vi "BIN_PAQ_Concat_PAQ_samples.vi"(7 "Memory TAGs":string[](array[string]), 8 "error in (no error)":errorcluster, 9 "Added samples TAGs":string[](array[string]), 10 "PAQ Samples to ADD":T1, 11 "PAQ Samples IN":T1) -> (0 "error out":errorcluster, 3 "PAQ Samples OUT":T1)   [LabVIEW 2020, in "Sgraph_lib_V1.lvlib" / "DBAL-BIN.lvclass"]
doc: "Andre Koelewijn, 7 mar 2021\n\nThis vi will concatenate PAQ samples based on a PAQ taglist of the samples as it is required for loading in FAMM memory. This routine will add the content based on newest data first. It will subsequenctly expect data chuncks going back in time for every iteration."
uses:
  DBAL-BIN.lvclass
  controls/BIN/BINdata.ctl
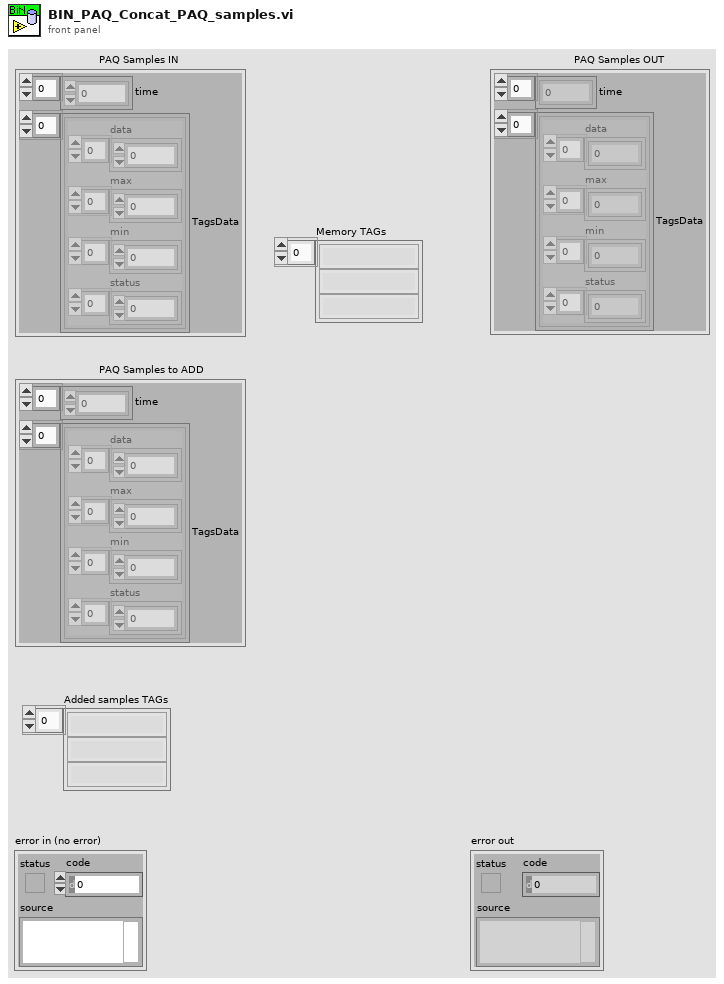
[diagram p1: front panel]
types:
  T1 = typedef "Sgraph_lib_V1.lvlib/DBAL-BIN.lvclass/BINdata.ctl" = cluster{"time":dbl[], "TagsData":cluster{"data":dbl[], "max":dbl[], "min":dbl[], "status":u32[]}[]}
  T2 = cluster{"data":dbl[], "max":dbl[], "min":dbl[], "status":u32[]}[]
  T3 = cluster{"data":dbl[], "max":dbl[], "min":dbl[], "status":u32[]}
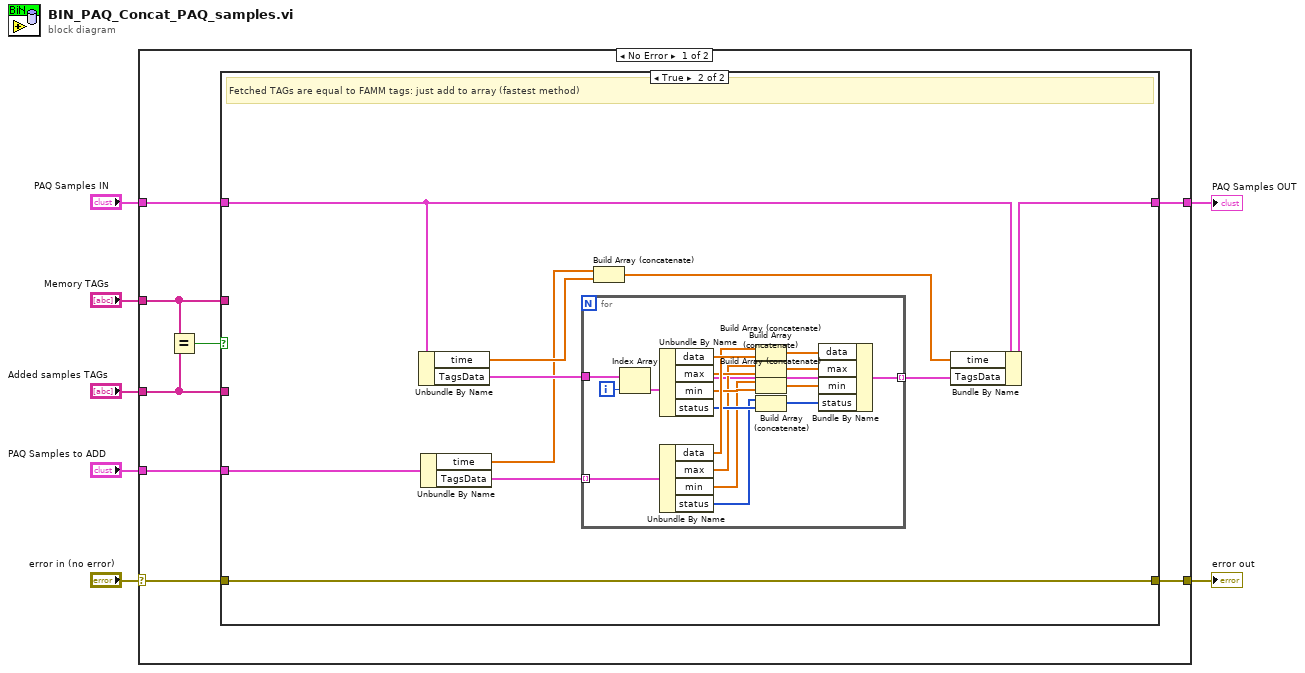
[diagram p0: block diagram]
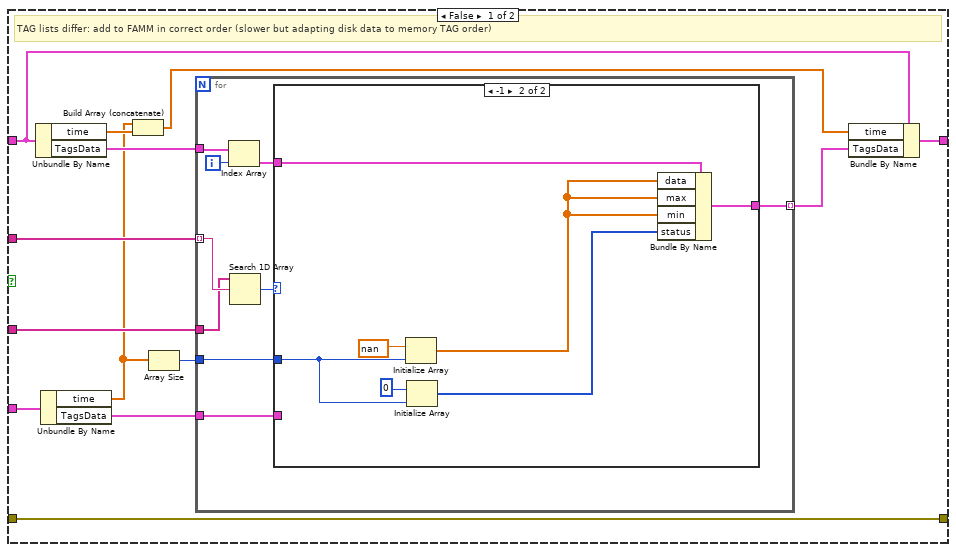
[diagram p2: hidden frame]
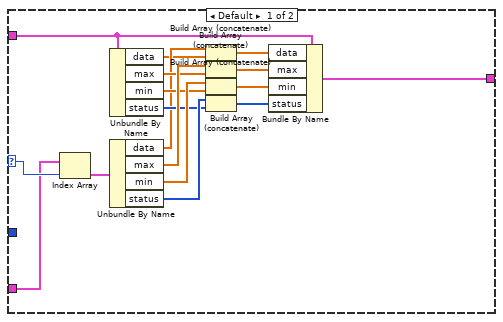
[diagram p3: hidden frame]
diagram:
  n1 = case shown="No Error" "error in (no error)" {
    selector: "error in (no error)" -> [w14 w90]
    tunnel: [w12 w90] -> w6
    tunnel: "PAQ Samples IN" -> [w15 w89]
    tunnel: [w13 w89] -> w4
    tunnel: "Memory TAGs" -> [w9 _]
    tunnel: "Added samples TAGs" -> [w10 _]
    tunnel: "PAQ Samples to ADD" -> [w11 _]
    frame No Error {
      n2 = Equal?(x=w9, y=w10) -> (x = y?=w8:bool)
      n3 = case shown="True" w8 {
        tunnel: w15 -> [w16 w63]
        tunnel: w14 -> [w28 w71]
        tunnel: [w17 w64] -> w13
        tunnel: [w28 w71] -> w12
        tunnel: w11 -> [w24 w62]
        tunnel: w10 -> [w27 _]
        tunnel: w9 -> [w26 _]
        frame False {
          # "TAG lists differ: add to FAMM in correct order (slower but adapting disk data to memory TAG order)"
          n4 = Unbundle By Name(w16) -> ("time"=w25:dbl[], "TagsData"=w22:T2)
          n5 = Unbundle By Name(w24) -> ("time"=w20:dbl[], "TagsData"=w18:T2)
          n6 = Build Array (concatenate)(w20, w25) -> (w23:dbl[])
          n7 = Array Size(array=w20) -> (size(s)=w19:i32)
          n8 = for {
            tunnel: w27 -> [w32]
            tunnel: w26 -> [w36] mode=indexing
            tunnel: w22 -> [w35]
            tunnel: [w31] -> w21 mode=indexing
            tunnel: w19 -> [w30]
            tunnel: w18 -> [w29]
            i -> [w34]
            n9 = Index Array(array=w35, index=w34) -> (element=w33:T3)
            n10 = Search 1D Array(1D array=w32, element=w36) -> (index of element=w37:i32)  [unwired: 1 in]
            n11 = case shown="-1" w37 {
              selector: w37 -> [w42 _]
              tunnel: w33 -> [w40 w60]
              tunnel: [w41 w61] -> w31
              tunnel: w30 -> [_ w57]
              tunnel: w29 -> [w39 _]
              frame Default {
                n12 = Index Array(array=w39, index=w42) -> (element=w38:T3)
                n13 = Unbundle By Name(w40) -> ("data"=w43:dbl[], "max"=w45:dbl[], "min"=w46:dbl[], "status"=w47:u32[])
                n14 = Unbundle By Name(w38) -> ("data"=w44:dbl[], "max"=w50:dbl[], "min"=w49:dbl[], "status"=w48:u32[])
                n15 = Build Array (concatenate)(w44, w43) -> (w53:dbl[])
                n16 = Build Array (concatenate)(w50, w45) -> (w52:dbl[])
                n17 = Build Array (concatenate)(w49, w46) -> (w51:dbl[])
                n18 = Build Array (concatenate)(w48, w47) -> (w54:u32[])
                n19 = Bundle By Name(cluster=w40, "data"=w53, "max"=w52, "min"=w51, "status"=w54) -> (w41:T3)
              }
              frame -1 {
                n20 = Initialize Array(nan ("value"), w57) -> (w58:dbl[])
                n21 = Initialize Array(u32 0 ("value"), w57) -> (w55:u32[])
                n22 = Bundle By Name(cluster=w60, "data"=w58, "max"=w58, "min"=w58, "status"=w55) -> (w61:T3)
              }
            }
          }
          n23 = Bundle By Name(cluster=w16, "time"=w23, "TagsData"=w21) -> (w17:T1)
        }
        frame True {
          # "Fetched TAGs are equal to FAMM tags: just add to array (fastest method)"
          n24 = Unbundle By Name(w63) -> ("time"=w66:dbl[], "TagsData"=w68:T2)
          n25 = Unbundle By Name(w62) -> ("time"=w65:dbl[], "TagsData"=w67:T2)
          n26 = for {
            tunnel: w67 -> [w86] mode=indexing
            tunnel: w68 -> [w88]
            tunnel: [w76] -> w69 mode=indexing
            i -> [w87]
            n27 = Index Array(array=w88, index=w87) -> (element=w77:T3)
            n28 = Unbundle By Name(w77) -> ("data"=w85:dbl[], "max"=w83:dbl[], "min"=w82:dbl[], "status"=w81:u32[])
            n29 = Unbundle By Name(w86) -> ("data"=w84:dbl[], "max"=w78:dbl[], "min"=w79:dbl[], "status"=w80:u32[])
            n30 = Build Array (concatenate)(w84, w85) -> (w73:dbl[])
            n31 = Build Array (concatenate)(w78, w83) -> (w74:dbl[])
            n32 = Build Array (concatenate)(w79, w82) -> (w75:dbl[])
            n33 = Build Array (concatenate)(w80, w81) -> (w72:u32[])
            n34 = Bundle By Name(cluster=w77, "data"=w73, "max"=w74, "min"=w75, "status"=w72) -> (w76:T3)
          }
          n35 = Build Array (concatenate)(w65, w66) -> (w70:dbl[])
          n36 = Bundle By Name(cluster=w63, "time"=w70, "TagsData"=w69) -> (w64:T1)
        }
      }
    }
    frame Error {
    }
  }
  "error out" <- w6
  "PAQ Samples OUT" <- w4
